vi "onSubscribe.vi"(6 "timeout (1000ms)":i32=1000, 8 "error in (no error)":errorcluster, 10 "SUBSCRIBE":refnum<class "SUBSCRIBE.lvclass">, 11 "Client in":refnum<class "Client.lvclass">) -> (0 "error out":errorcluster, 1 "Ack?":bool, 2 "SUBACK":refnum<class "SUBACK.lvclass">, 3 "Client out":refnum<class "Client.lvclass">)   [LabVIEW 2013, in "MQTT Client.lvlib" / "Client.lvclass"]
uses:
  Client.lvclass
  <vilib>/LabVIEW Open Source Project/MQTT Control Packets/Control Packets/SUBSCRIBE/SUBSCRIBE.lvclass
  <vilib>/LabVIEW Open Source Project/MQTT Control Packets/Control Packets/SUBACK/SUBACK.lvclass
  <vilib>/LabVIEW Open Source Project/MQTT Control Packets/Control Packets/ControlPacket/ControlPacket.lvclass/ControlPacket.ctl
  Session.Client/Session.Client.lvclass
  <vilib>/LabVIEW Open Source Project/MQTT Control Packets/Control Packets/ControlPacket/ControlPacket.lvclass
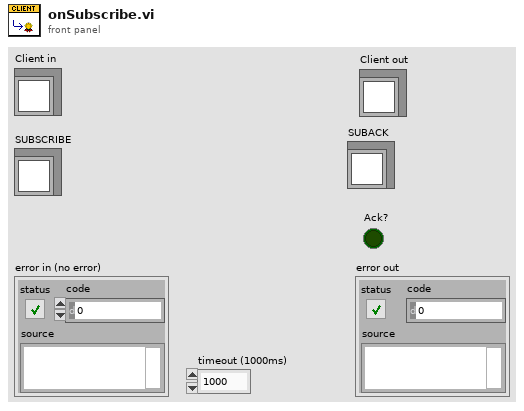
[diagram p1: front panel]
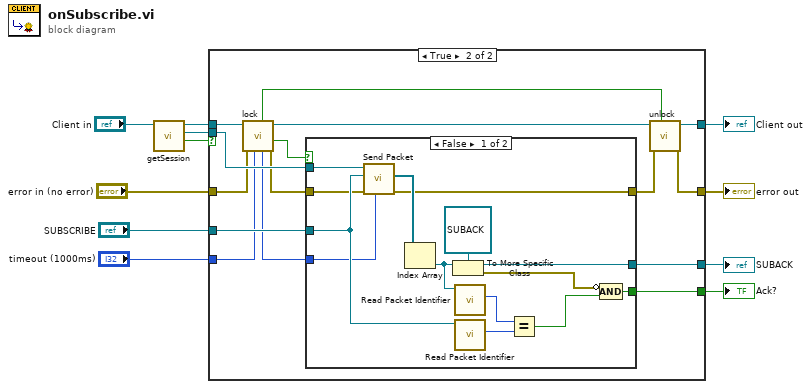
[diagram p0: block diagram]
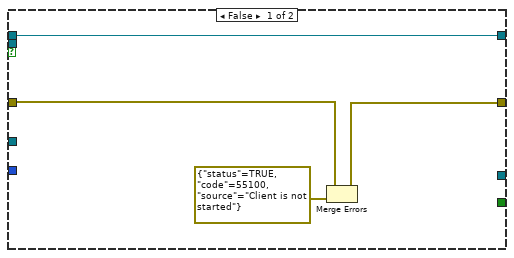
[diagram p2: hidden frame]
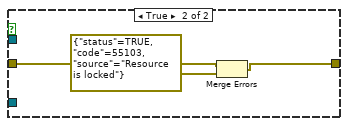
[diagram p3: hidden frame]
diagram:
  n1 = call "getSession.vi"("Client in"="Client in") -> ("valid?"=w7:bool, "Session"=w6:refnum<class "Session.Client.lvclass">, "Client out"=w8:refnum<class "Client.lvclass">)  [unwired: 8 in]
  n2 = case shown="True" w7 {
    tunnel: [w12 w24] -> w5
    tunnel: "error in (no error)" -> [w14 w21]
    tunnel: [w13 w17] -> w4
    tunnel: "timeout (1000ms)" -> [_ w23]
    tunnel: [_ w30] -> w11
    tunnel: "SUBSCRIBE" -> [_ w29]
    tunnel: [_ w28] -> w9
    tunnel: w8 -> [w12 w26]
    tunnel: w6 -> [_ w27]
    frame False {
      n3 = Merge Errors(w14, errorcluster {"status"=TRUE, "code"=55100, "source"="Client is not started"} ("error in")) -> (w13:errorcluster)
    }
    frame True {
      n4 = call "lock.vi"("timeout (2000ms)"=w23, "error in (no error)"=w21, "Client in"=w26) -> ("error out"=w20:errorcluster, "timed out"=w16:bool, "Client out"=w25:refnum<class "Client.lvclass">, "remaining (ms)"=w22:i32, "locked"=w19:bool)  [unwired: 4 in]
      n5 = case shown="False" w16 {
        tunnel: [w43 _] -> w30
        tunnel: w29 -> [w41 _]
        tunnel: [w36 _] -> w28
        tunnel: w27 -> [w35 _]
        tunnel: w22 -> [w33 _]
        tunnel: w20 -> [w32 w46]
        tunnel: [w31 w45] -> w18
        frame False {
          n6 = call "Send Packet.vi"("timeout (0ms : no ack)"=w33, "error in (no error)"=w32, "Packet"=w41, "Session"=w35) -> ("error out"=w31:errorcluster, "Response"=w44:refnum<class "ControlPacket.lvclass">[])  [unwired: 4 in, 2 out]
          n7 = Index Array(array=w44) -> (element=w40:refnum<class "ControlPacket.lvclass">)  [unwired: 1 in]
          n8 = To More Specific Class(target class=refnum<class "SUBACK.lvclass"> refnum ("SUBACK.lvclass"), reference=w40) -> (specific class reference=w43:refnum<class "SUBACK.lvclass">, error out=w37:errorcluster)  [unwired: 1 in]
          n9 = call <vilib>:"Read Packet Identifier.vi"("ControlPacket in"=w40) -> ("Packet Identifier"=w39:u16)  [unwired: 9 in, 1 out]
          n10 = call <vilib>:"Read Packet Identifier.vi"("ControlPacket in"=w41) -> ("Packet Identifier"=w38:u16)  [unwired: 9 in, 1 out]
          n11 = Equal?(x=w39, y=w38) -> (x = y?=w34:bool)
          n12 = Compound Arithmetic op=AND(invert w37, w34) -> (w36:bool)
        }
        frame True {
          n13 = Merge Errors(w46, errorcluster {"status"=TRUE, "code"=55103, "source"="Resource is locked"} ("error in")) -> (w45:errorcluster)
        }
      }
      n14 = call "unlock.vi"("Unlock?"=w19, "error in (no error)"=w18, "Client in"=w25) -> ("error out"=w17:errorcluster, "Client out"=w24:refnum<class "Client.lvclass">)  [unwired: 7 in]
    }
  }
  "error out" <- w4
  "Client out" <- w5
  "SUBACK" <- w11
  "Ack?" <- w9
